vi "Create_Stop_Event.vi"(8 "error in (no error)":errorcluster={"status"=FALSE, "code"=0, "source"="\"\""}) -> (0 "error out":errorcluster, 3 "User Event - Stop":refnum<user-event>)   [LabVIEW 2026]
doc: "Create a boolean user event to stop parallel loops."
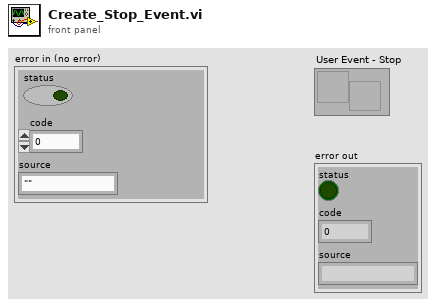
[diagram p1: front panel]
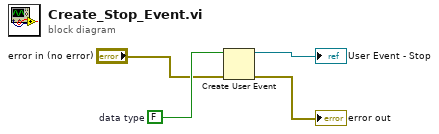
[diagram p0: block diagram]
diagram:
  w2 = FALSE  # data type
  n1 = Create User Event(user event datatype=w2, error in="error in (no error)") -> (user event=→"User Event - Stop":refnum<user-event>, error out=→"error out":errorcluster)
